vi "Alarm_Battery.vi"   [LabVIEW 2025]
panel:
  # "CANH BAO!!!\nPIN HOAT DONG YEU!!!\nVUI LONG THAY THE PIN MOI VA CHAY KIEM TRA LAI"
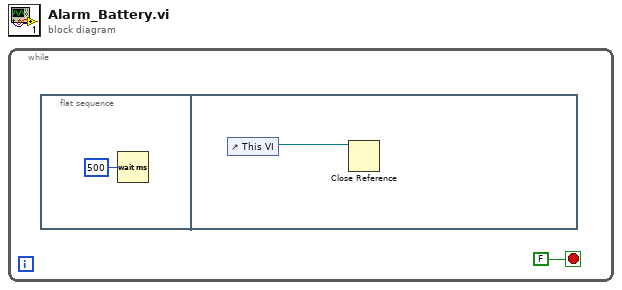
[diagram p0: block diagram]
diagram:
  n1 = while {
    stop <- FALSE stop-if-true
    n2 = flat-sequence {
      frame #0 {
        n3 = Wait (ms)(milliseconds to wait=u32 500) -> ()  [unwired: 1 out]
      }
      frame #1 {
        n4 = control-ref of="This VI"() -> (w3:refnum<vi>)
        n5 = Close Reference(reference=w3) -> ()  [unwired: 1 in, 1 out]
      }
    }
  }
